vi "run iterator.vi"(8 "error in (no error)":errorcluster, 11 "SPARC4_GEI in":refnum<class "S4GEI.lvclass">) -> (0 "error out":errorcluster, 3 "SPARC4_GEI out":refnum<class "S4GEI.lvclass">)   [LabVIEW 2018, in "S4GEI.lvclass"]
uses:
  S4GEI.lvclass
  FWCS_ACS_Iterator/FWCS_ACS_Iterator.lvclass
  Filter_Wheel/Filter_Wheel.lvclass
  Channel GUI/Channel.lvclass
  Camera/Camera.lvclass
panel:
  in  "Filter":u16(ring) items=["U"=1, "B"=2, "V"=3, "R"=4, "I"=5, "Clear"=6]
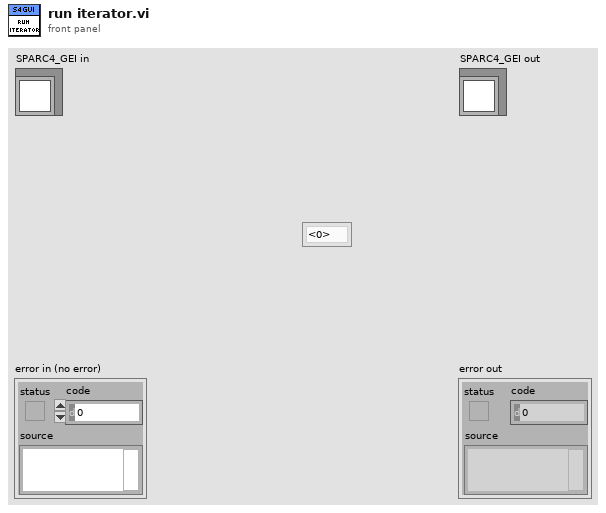
[diagram p1: front panel]
types:
  T1 = cluster{"Select":bool, "Exp Time":dbl, "#Frames":u16, "Sufix":string, "Filter":u16}[]
  T2 = cluster{"Select":bool, "Exp Time":dbl, "#Frames":u16, "Sufix":string, "Filter":u16}
  T3 = cluster{"COOLER_POWER_STATUS":u16, "TEMP":i32, "EXPTIME":dbl, "#FRAMES":u32, "#CYCLES":u32, "#SEQS":u32, "WAVEPLATE_POS":u16, "suffix":string}
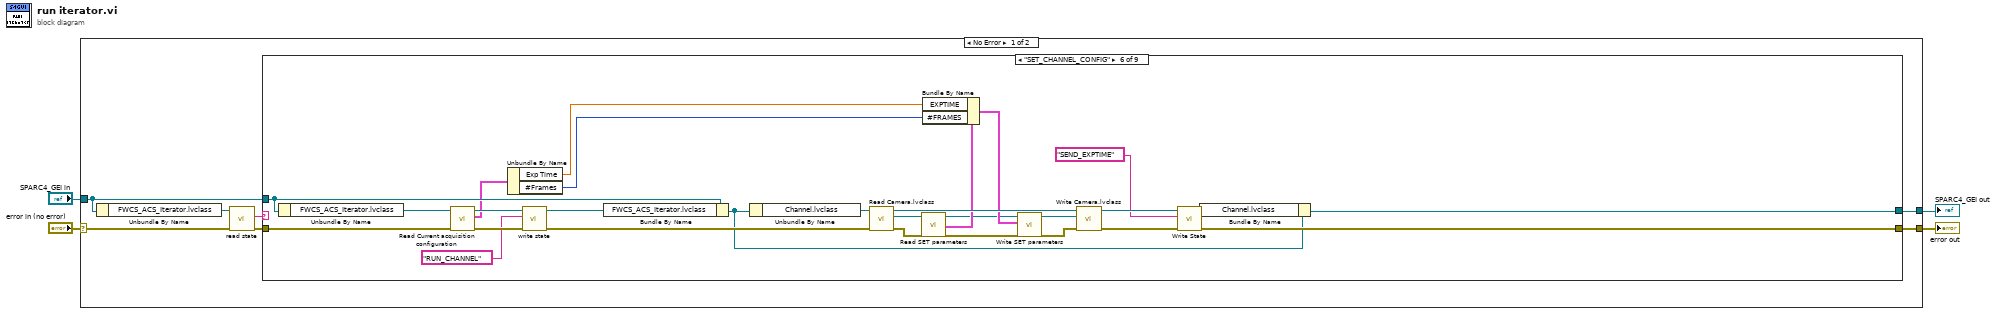
[diagram p0: block diagram]
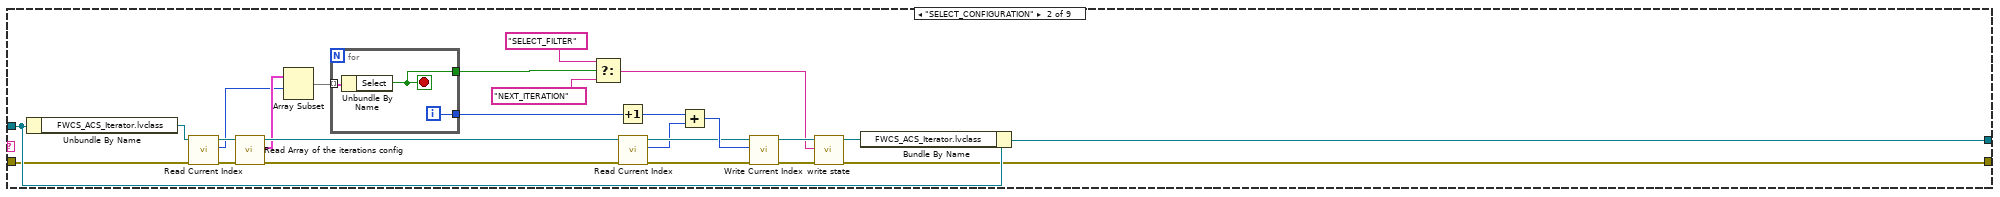
[diagram p3: hidden frame]
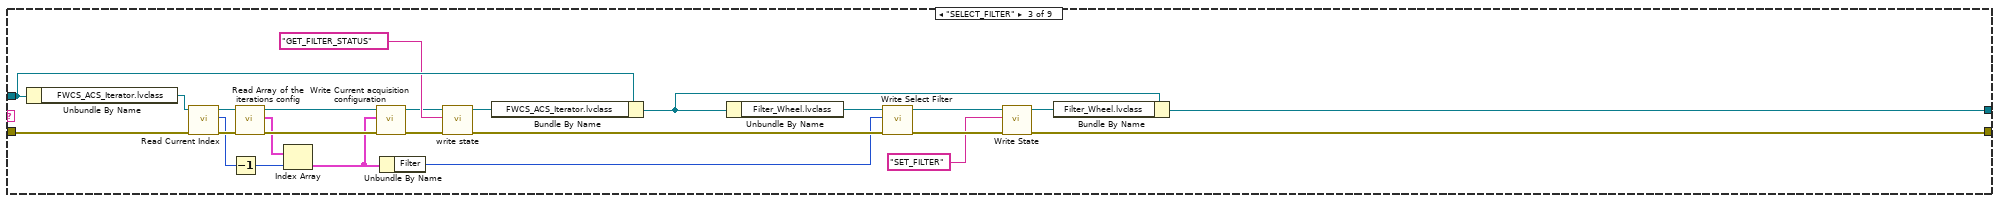
[diagram p4: hidden frame]
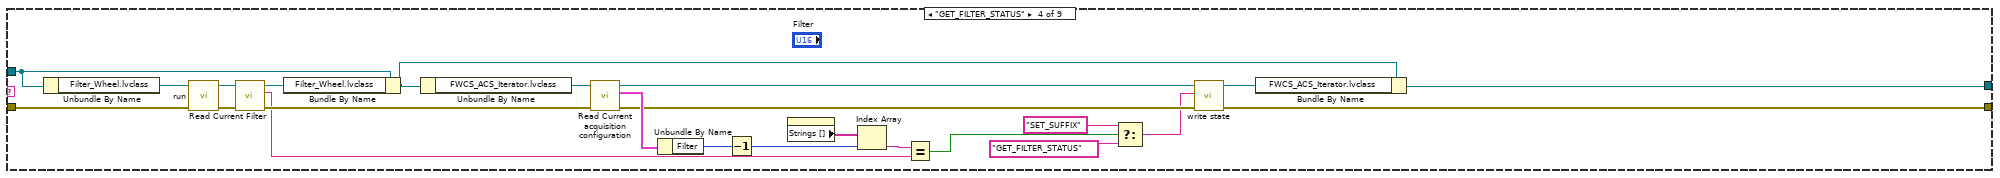
[diagram p5: hidden frame]
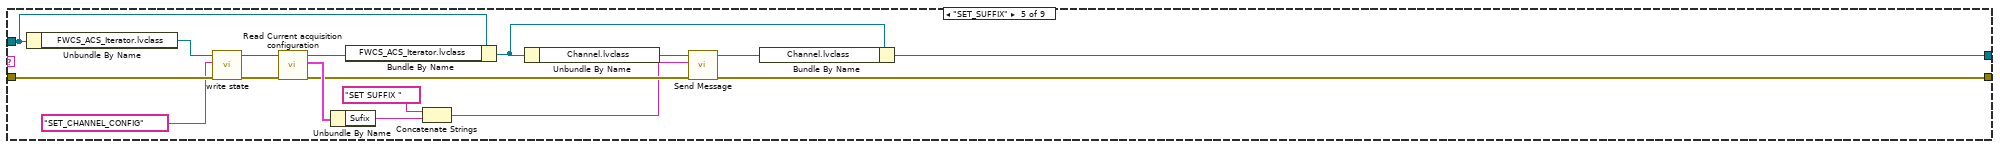
[diagram p6: hidden frame]
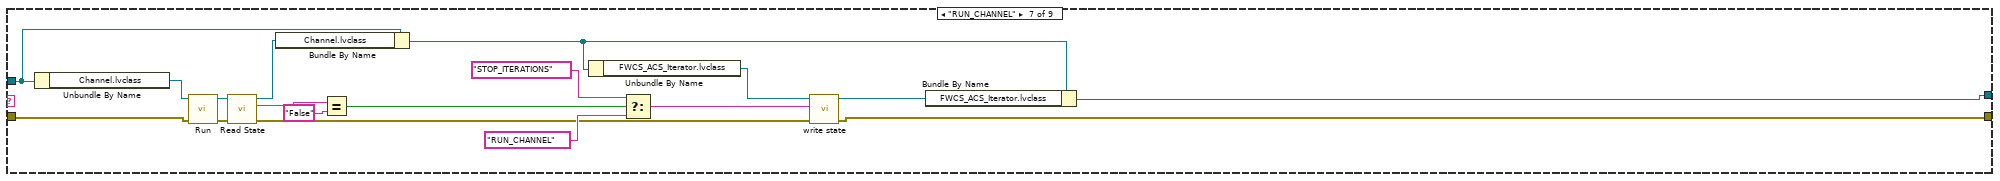
[diagram p7: hidden frame]
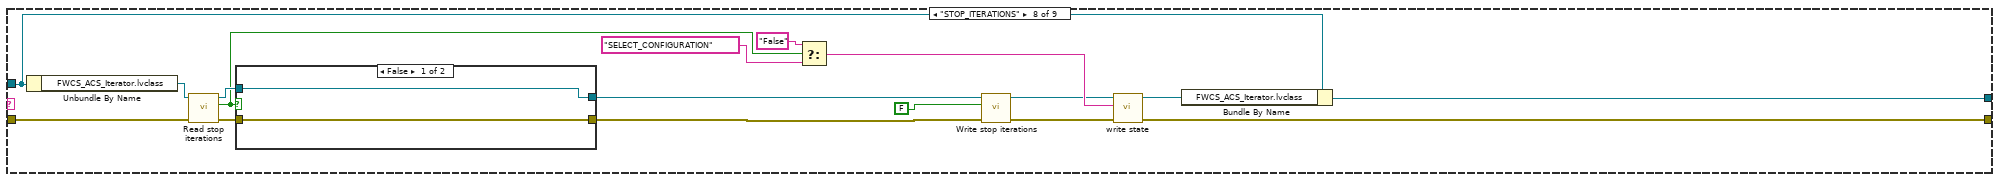
[diagram p8: hidden frame]
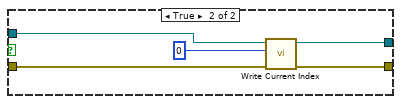
[diagram p9: hidden frame]
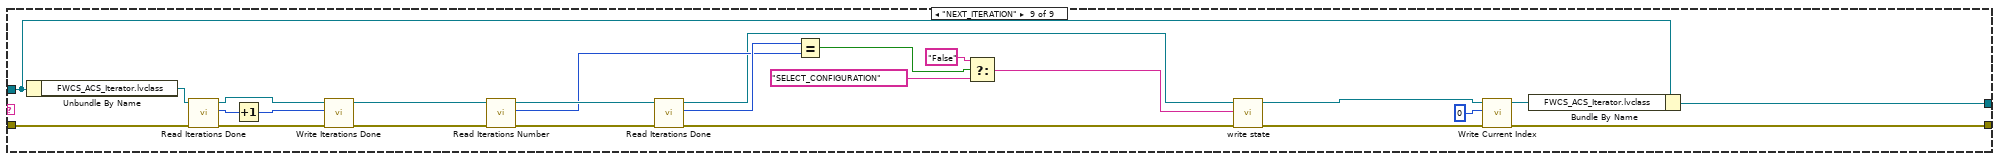
[diagram p10: hidden frame]
diagram:
  n1 = case shown="No Error" "error in (no error)" {
    selector: "error in (no error)" -> [w10 w204]
    tunnel: [w5 w204] -> w3
    tunnel: [w6 w203] -> w1
    tunnel: "SPARC4_GEI in" -> [w8 w203]
    frame No Error {
      n2 = Unbundle By Name(w8) -> ("FWCS_ACS_Iterator.lvclass"=w11:refnum<class "FWCS_ACS_Iterator.lvclass">)
      n3 = call "read state.vi"("error in (no error)"=w10, "FWCS_ACS_Iterator in"=w11) -> ("error out"=w7:errorcluster, "State"=w9:string)  [unwired: 7 in, 1 out]
      n4 = case shown="\"SET_CHANNEL_CONFIG\"" w9 {
        tunnel: w8 -> [w13 w36 w66 w86 w100 w125 w153 w169 w201]
        tunnel: w7 -> [w12 w31 w60 w90 w103 w134 w137 w162 w186]
        tunnel: [w13 w35 w47 w73 w94 w131 w143 w170 w202] -> w6
        tunnel: [w12 w24 w46 w74 w93 w130 w144 w165 w182] -> w5
        frame "False", Default {
        }
        frame "SELECT_CONFIGURATION" {
          n5 = Unbundle By Name(w36) -> ("FWCS_ACS_Iterator.lvclass"=w32:refnum<class "FWCS_ACS_Iterator.lvclass">)
          n6 = call "Read Current Index.vi"("error in (no error)"=w31, "FWCS_ACS_Iterator in"=w32) -> ("error out"=w34:errorcluster, "Current Index"=w26:u16, "FWCS_ACS_Iterator out"=w33:refnum<class "FWCS_ACS_Iterator.lvclass">)  [unwired: 7 in]
          n7 = call "Read Array of the iterations config.vi"("error in (no error)"=w34, "FWCS_ACS_Iterator in"=w33) -> ("error out"=w37:errorcluster, "Array of the iterations config"=w30:T1, "FWCS_ACS_Iterator out"=w38:refnum<class "FWCS_ACS_Iterator.lvclass">)  [unwired: 7 in]
          n8 = Array Subset(array=w30, index=w26) -> (w29:T1)  [unwired: 1 in]
          n9 = for {
            tunnel: w29 -> [w41] mode=indexing
            tunnel: [w40] -> w15
            tunnel: [w39] -> w19
            i -> [w40]
            stop <- w39 stop-if-true
            n10 = Unbundle By Name(w41) -> ("Select"=w39:bool)
          }
          n11 = Select(t="SELECT_FILTER", s=w19, f="NEXT_ITERATION") -> (s? t:f=w16:string)
          n12 = Increment(x=w15) -> (x+1=w14:i32)
          n13 = call "Read Current Index.vi"("error in (no error)"=w37, "FWCS_ACS_Iterator in"=w38) -> ("error out"=w23:errorcluster, "Current Index"=w21:u16, "FWCS_ACS_Iterator out"=w22:refnum<class "FWCS_ACS_Iterator.lvclass">)  [unwired: 7 in]
          n14 = Add(x=w14, y=w21) -> (x+y=w25:i32)
          n15 = call "Write Current Index.vi"("error in (no error)"=w23, "Current Index"=w25, "FWCS_ACS_Iterator in"=w22) -> ("error out"=w27:errorcluster, "FWCS_ACS_Iterator out"=w28:refnum<class "FWCS_ACS_Iterator.lvclass">)  [unwired: 7 in]
          n16 = call "write state.vi"("error in (no error)"=w27, "State"=w16, "FWCS_ACS_Iterator in"=w28) -> ("error out"=w24:errorcluster, "FWCS_ACS_Iterator out"=w20:refnum<class "FWCS_ACS_Iterator.lvclass">)  [unwired: 7 in]
          n17 = Bundle By Name(cluster=w36, "FWCS_ACS_Iterator.lvclass"=w20) -> (w35:refnum<class "S4GEI.lvclass">)
        }
        frame "SELECT_FILTER" {
          n18 = Unbundle By Name(w66) -> ("FWCS_ACS_Iterator.lvclass"=w61:refnum<class "FWCS_ACS_Iterator.lvclass">)
          n19 = call "Read Current Index.vi"("error in (no error)"=w60, "FWCS_ACS_Iterator in"=w61) -> ("error out"=w59:errorcluster, "Current Index"=w54:u16, "FWCS_ACS_Iterator out"=w58:refnum<class "FWCS_ACS_Iterator.lvclass">)  [unwired: 7 in]
          n20 = Decrement(x=w54) -> (x-1=w53:u16)
          n21 = call "Read Array of the iterations config.vi"("error in (no error)"=w59, "FWCS_ACS_Iterator in"=w58) -> ("error out"=w57:errorcluster, "Array of the iterations config"=w55:T1, "FWCS_ACS_Iterator out"=w56:refnum<class "FWCS_ACS_Iterator.lvclass">)  [unwired: 7 in]
          n22 = Index Array(array=w55, index=w53) -> (element=w43:T2)
          n23 = call "Write Current acquisition configuration.vi"("error in (no error)"=w57, "Current acquisition configuration"=w43, "FWCS_ACS_Iterator in"=w56) -> ("error out"=w62:errorcluster, "FWCS_ACS_Iterator out"=w63:refnum<class "FWCS_ACS_Iterator.lvclass">)  [unwired: 7 in]
          n24 = Unbundle By Name(w43) -> ("Filter"=w42:u16)
          n25 = call "write state.vi"("error in (no error)"=w62, "State"="GET_FILTER_STATUS", "FWCS_ACS_Iterator in"=w63) -> ("error out"=w44:errorcluster, "FWCS_ACS_Iterator out"=w64:refnum<class "FWCS_ACS_Iterator.lvclass">)  [unwired: 7 in]
          n26 = Bundle By Name(cluster=w66, "FWCS_ACS_Iterator.lvclass"=w64) -> (w49:refnum<class "S4GEI.lvclass">)
          n27 = Unbundle By Name(w49) -> ("Filter_Wheel.lvclass"=w50:refnum<class "Filter_Wheel.lvclass">)
          n28 = call "Write Select Filter.vi"("error in (no error)"=w44, "Select Filter"=w42, "Filter_Wheel in"=w50) -> ("error out"=w52:errorcluster, "Filter_Wheel out"=w45:refnum<class "Filter_Wheel.lvclass">)  [unwired: 7 in]
          n29 = call "Write State.vi"("error in (no error)"=w52, "State"="SET_FILTER", "Filter_Wheel in"=w45) -> ("error out"=w46:errorcluster, "Filter_Wheel out"=w48:refnum<class "Filter_Wheel.lvclass">)  [unwired: 7 in]
          n30 = Bundle By Name(cluster=w49, "Filter_Wheel.lvclass"=w48) -> (w47:refnum<class "S4GEI.lvclass">)
        }
        frame "GET_FILTER_STATUS" {
          n31 = Unbundle By Name(w86) -> ("Filter_Wheel.lvclass"=w89:refnum<class "Filter_Wheel.lvclass">)
          n32 = call "run.vi"("error in (no error)"=w90, "Filter_Wheel in"=w89) -> ("error out"=w88:errorcluster, "Filter_Wheel out"=w87:refnum<class "Filter_Wheel.lvclass">)  [unwired: 8 in]
          n33 = call "Read Current Filter.vi"("error in (no error)"=w88, "Filter_Wheel in"=w87) -> ("error out"=w82:errorcluster, "Current Filter"=w78:string, "Filter_Wheel out"=w85:refnum<class "Filter_Wheel.lvclass">)  [unwired: 7 in]
          n34 = Bundle By Name(cluster=w86, "Filter_Wheel.lvclass"=w85) -> (w84:refnum<class "S4GEI.lvclass">)
          n35 = Unbundle By Name(w84) -> ("FWCS_ACS_Iterator.lvclass"=w83:refnum<class "FWCS_ACS_Iterator.lvclass">)
          n36 = call "Read Current acquisition configuration.vi"("error in (no error)"=w82, "FWCS_ACS_Iterator in"=w83) -> ("error out"=w77:errorcluster, "Current acquisition configuration"=w81:T2, "FWCS_ACS_Iterator out"=w76:refnum<class "FWCS_ACS_Iterator.lvclass">)  [unwired: 7 in]
          n37 = Unbundle By Name(w81) -> ("Filter"=w68:u16)
          n38 = Decrement(x=w68) -> (x-1=w67:u16)
          n39 = property on="Filter" class="Ring (strict)"() -> ("Strings []"=w80:string[])  [unwired: 2 in, 2 out]
          n40 = Index Array(array=w80, index=w67) -> (element=w79:string)
          n41 = Equal?(x=w79, y=w78) -> (x = y?=w72:bool)
          n42 = Select(t="SET_SUFFIX", s=w72, f="GET_FILTER_STATUS") -> (s? t:f=w69:string)
          n43 = call "write state.vi"("error in (no error)"=w77, "State"=w69, "FWCS_ACS_Iterator in"=w76) -> ("error out"=w74:errorcluster, "FWCS_ACS_Iterator out"=w75:refnum<class "FWCS_ACS_Iterator.lvclass">)  [unwired: 7 in]
          n44 = Bundle By Name(cluster=w84, "FWCS_ACS_Iterator.lvclass"=w75) -> (w73:refnum<class "S4GEI.lvclass">)
        }
        frame "SET_SUFFIX" {
          n45 = Unbundle By Name(w100) -> ("FWCS_ACS_Iterator.lvclass"=w104:refnum<class "FWCS_ACS_Iterator.lvclass">)
          n46 = call "write state.vi"("error in (no error)"=w103, "State"="SET_CHANNEL_CONFIG", "FWCS_ACS_Iterator in"=w104) -> ("error out"=w101:errorcluster, "FWCS_ACS_Iterator out"=w102:refnum<class "FWCS_ACS_Iterator.lvclass">)  [unwired: 7 in]
          n47 = call "Read Current acquisition configuration.vi"("error in (no error)"=w101, "FWCS_ACS_Iterator in"=w102) -> ("error out"=w97:errorcluster, "Current acquisition configuration"=w107:T2, "FWCS_ACS_Iterator out"=w99:refnum<class "FWCS_ACS_Iterator.lvclass">)  [unwired: 7 in]
          n48 = Unbundle By Name(w107) -> ("Sufix"=w95:string)
          n49 = Bundle By Name(cluster=w100, "FWCS_ACS_Iterator.lvclass"=w99) -> (w98:refnum<class "S4GEI.lvclass">)
          n50 = Concatenate Strings("SET SUFFIX ", w95) -> (w91:string)
          n51 = Unbundle By Name(w98) -> ("Channel.lvclass"=w106:refnum<class "Channel.lvclass">)
          n52 = call "Send Message.vi"("error in (no error)"=w97, "Message"=w91, "Channel GUI in"=w106) -> ("error out"=w93:errorcluster, "Channel GUI out"=w105:refnum<class "Channel.lvclass">)  [unwired: 7 in]
          n53 = Bundle By Name(cluster=w98, "Channel.lvclass"=w105) -> (w94:refnum<class "S4GEI.lvclass">)
        }
        frame "SET_CHANNEL_CONFIG" {
          n54 = Unbundle By Name(w125) -> ("FWCS_ACS_Iterator.lvclass"=w135:refnum<class "FWCS_ACS_Iterator.lvclass">)
          n55 = call "Read Current acquisition configuration.vi"("error in (no error)"=w134, "FWCS_ACS_Iterator in"=w135) -> ("error out"=w129:errorcluster, "Current acquisition configuration"=w122:T2, "FWCS_ACS_Iterator out"=w128:refnum<class "FWCS_ACS_Iterator.lvclass">)  [unwired: 7 in]
          n56 = Unbundle By Name(w122) -> ("Exp Time"=w112:dbl, "#Frames"=w111:u16)
          n57 = call "write state.vi"("error in (no error)"=w129, "State"="RUN_CHANNEL", "FWCS_ACS_Iterator in"=w128) -> ("error out"=w127:errorcluster, "FWCS_ACS_Iterator out"=w123:refnum<class "FWCS_ACS_Iterator.lvclass">)  [unwired: 7 in]
          n58 = Bundle By Name(cluster=w125, "FWCS_ACS_Iterator.lvclass"=w123) -> (w124:refnum<class "S4GEI.lvclass">)
          n59 = Unbundle By Name(w124) -> ("Channel.lvclass"=w133:refnum<class "Channel.lvclass">)
          n60 = call-dynamic "Read Camera.lvclass.vi"("error in (no error)"=w127, "Channel in"=w133) -> ("error out"=w119:errorcluster, "Camera.lvclass"=w120:refnum<class "Camera.lvclass">, "Channel out"=w121:refnum<class "Channel.lvclass">)  [unwired: 7 in]
          n61 = call-dynamic "Read SET parameters.vi"("error in (no error)"=w119, "Camera in"=w120) -> ("error out"=w118:errorcluster, "SET parameters"=w110:T3, "Camera out"=w109:refnum<class "Camera.lvclass">)  [unwired: 7 in]
          n62 = Bundle By Name(cluster=w110, "EXPTIME"=w112, "#FRAMES"=w111) -> (w116:T3)
          n63 = call-dynamic "Write SET parameters.vi"("error in (no error)"=w118, "SET parameters"=w116, "Camera in"=w109) -> ("error out"=w117:errorcluster, "Camera out"=w108:refnum<class "Camera.lvclass">)  [unwired: 7 in]
          n64 = call-dynamic "Write Camera.lvclass.vi"("error in (no error)"=w117, "Camera.lvclass"=w108, "Channel in"=w121) -> ("error out"=w115:errorcluster, "Channel out"=w114:refnum<class "Channel.lvclass">)  [unwired: 7 in]
          n65 = call "Write State.vi"("error in (no error)"=w115, "State"="SEND_EXPTIME", "Channel GEI in"=w114) -> ("error out"=w130:errorcluster, "Channel GEI out"=w132:refnum<class "Channel.lvclass">)  [unwired: 7 in]
          n66 = Bundle By Name(cluster=w124, "Channel.lvclass"=w132) -> (w131:refnum<class "S4GEI.lvclass">)
        }
        frame "RUN_CHANNEL" {
          n67 = Unbundle By Name(w153) -> ("Channel.lvclass"=w136:refnum<class "Channel.lvclass">)
          n68 = call "Run.vi"("error in (no error)"=w137, "Channel GUI in"=w136) -> ("error out"=w138:errorcluster, "Channel GUI out"=w142:refnum<class "Channel.lvclass">)  [unwired: 8 in]
          n69 = call "Read State.vi"("error in (no error)"=w138, "Channel GEI in"=w142) -> ("error out"=w139:errorcluster, "State"=w140:string, "Channel GEI out"=w141:refnum<class "Channel.lvclass">)  [unwired: 7 in]
          n70 = Bundle By Name(cluster=w153, "Channel.lvclass"=w141) -> (w152:refnum<class "S4GEI.lvclass">)
          n71 = Equal?(x=w140, y="False") -> (x = y?=w148:bool)
          n72 = Unbundle By Name(w152) -> ("FWCS_ACS_Iterator.lvclass"=w151:refnum<class "FWCS_ACS_Iterator.lvclass">)
          n73 = Select(t="STOP_ITERATIONS", s=w148, f="RUN_CHANNEL") -> (s? t:f=w145:string)
          n74 = call "write state.vi"("error in (no error)"=w139, "State"=w145, "FWCS_ACS_Iterator in"=w151) -> ("error out"=w144:errorcluster, "FWCS_ACS_Iterator out"=w150:refnum<class "FWCS_ACS_Iterator.lvclass">)  [unwired: 7 in]
          n75 = Bundle By Name(cluster=w152, "FWCS_ACS_Iterator.lvclass"=w150) -> (w143:refnum<class "S4GEI.lvclass">)
        }
        frame "STOP_ITERATIONS" {
          n76 = Unbundle By Name(w169) -> ("FWCS_ACS_Iterator.lvclass"=w163:refnum<class "FWCS_ACS_Iterator.lvclass">)
          n77 = call "Read stop iterations.vi"("error in (no error)"=w162, "FWCS_ACS_Iterator in"=w163) -> ("error out"=w155:errorcluster, "stop iterations"=w154:bool, "FWCS_ACS_Iterator out"=w158:refnum<class "FWCS_ACS_Iterator.lvclass">)  [unwired: 7 in]
          n78 = case shown="False" w154 {
            tunnel: w158 -> [w172 w176]
            tunnel: [w172 w175] -> w157
            tunnel: [w171 w174] -> w156
            tunnel: w155 -> [w171 w173]
            frame False {
            }
            frame True {
              n79 = call "Write Current Index.vi"("error in (no error)"=w173, "Current Index"=u16 0, "FWCS_ACS_Iterator in"=w176) -> ("error out"=w174:errorcluster, "FWCS_ACS_Iterator out"=w175:refnum<class "FWCS_ACS_Iterator.lvclass">)  [unwired: 7 in]
            }
          }
          n80 = Select(t="False", s=w154, f="SELECT_CONFIGURATION") -> (s? t:f=w166:string)
          n81 = call "Write stop iterations.vi"("error in (no error)"=w156, "stop iterations"=FALSE, "FWCS_ACS_Iterator in"=w157) -> ("error out"=w161:errorcluster, "FWCS_ACS_Iterator out"=w160:refnum<class "FWCS_ACS_Iterator.lvclass">)  [unwired: 7 in]
          n82 = call "write state.vi"("error in (no error)"=w161, "State"=w166, "FWCS_ACS_Iterator in"=w160) -> ("error out"=w165:errorcluster, "FWCS_ACS_Iterator out"=w164:refnum<class "FWCS_ACS_Iterator.lvclass">)  [unwired: 7 in]
          n83 = Bundle By Name(cluster=w169, "FWCS_ACS_Iterator.lvclass"=w164) -> (w170:refnum<class "S4GEI.lvclass">)
        }
        frame "NEXT_ITERATION" {
          n84 = Unbundle By Name(w201) -> ("FWCS_ACS_Iterator.lvclass"=w187:refnum<class "FWCS_ACS_Iterator.lvclass">)
          n85 = call "Read Iterations Done.vi"("error in (no error)"=w186, "FWCS_ACS_Iterator in"=w187) -> ("error out"=w191:errorcluster, "Iterations Done"=w189:u16, "FWCS_ACS_Iterator out"=w190:refnum<class "FWCS_ACS_Iterator.lvclass">)  [unwired: 7 in]
          n86 = Increment(x=w189) -> (x+1=w188:u16)
          n87 = call "Write Iterations Done.vi"("error in (no error)"=w191, "Iterations Done"=w188, "FWCS_ACS_Iterator in"=w190) -> ("error out"=w184:errorcluster, "FWCS_ACS_Iterator out"=w185:refnum<class "FWCS_ACS_Iterator.lvclass">)  [unwired: 7 in]
          n88 = call "Read Iterations Number.vi"("error in (no error)"=w184, "FWCS_ACS_Iterator in"=w185) -> ("error out"=w200:errorcluster, "Iterations Number"=w197:u16, "FWCS_ACS_Iterator out"=w199:refnum<class "FWCS_ACS_Iterator.lvclass">)  [unwired: 7 in]
          n89 = call "Read Iterations Done.vi"("error in (no error)"=w200, "FWCS_ACS_Iterator in"=w199) -> ("error out"=w192:errorcluster, "Iterations Done"=w198:u16, "FWCS_ACS_Iterator out"=w193:refnum<class "FWCS_ACS_Iterator.lvclass">)  [unwired: 7 in]
          n90 = Equal?(x=w198, y=w197) -> (x = y?=w179:bool)
          n91 = Select(t="False", s=w179, f="SELECT_CONFIGURATION") -> (s? t:f=w194:string)
          n92 = call "write state.vi"("error in (no error)"=w192, "State"=w194, "FWCS_ACS_Iterator in"=w193) -> ("error out"=w183:errorcluster, "FWCS_ACS_Iterator out"=w180:refnum<class "FWCS_ACS_Iterator.lvclass">)  [unwired: 7 in]
          n93 = call "Write Current Index.vi"("error in (no error)"=w183, "Current Index"=u16 0, "FWCS_ACS_Iterator in"=w180) -> ("error out"=w182:errorcluster, "FWCS_ACS_Iterator out"=w181:refnum<class "FWCS_ACS_Iterator.lvclass">)  [unwired: 7 in]
          n94 = Bundle By Name(cluster=w201, "FWCS_ACS_Iterator.lvclass"=w181) -> (w202:refnum<class "S4GEI.lvclass">)
        }
      }
    }
    frame Error {
    }
  }
  "error out" <- w3
  "SPARC4_GEI out" <- w1
